vi "Host_Runtime_Monitor.vi"(8 "error in (no error)":errorcluster={"status"=FALSE, "code"=0, "source"="\"\""}, 10 "run identity":string, 11 "Incoming status/events":string) -> (0 "error out":errorcluster={"status"=FALSE, "code"=0, "source"="\"\""}, 2 "status ok":bool, 3 "HMI indicators":string)   [LabVIEW 2026]
doc: "INTENT: Display current execution. LOGIC: Update state, current group, active steps, cycle counts and fault details from event messages."
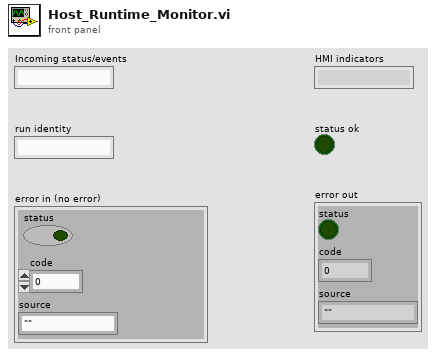
[diagram p1: front panel]
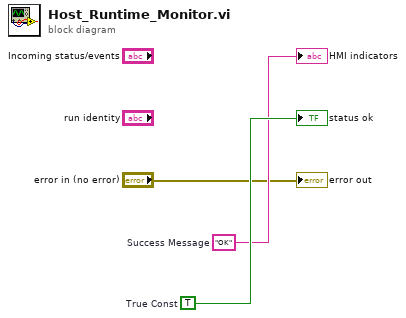
[diagram p0: block diagram]
diagram:
  w3 = TRUE  # True Const
  w2 = "OK"  # Success Message
  "HMI indicators" <- w2
  "status ok" <- w3
  "error out" <- "error in (no error)"
